vi "Read_Pong.vi"(8 "error in (no error)":errorcluster, 9 "rx state":T1, 10 "result":T2, 11 "TLS connection":refnum<k5>) -> (0 "error out":errorcluster)   [LabVIEW 2021, in "CANsub_API.lvlib"]
doc: "API private: sends a WebSocket pong (opcode 10, same payload) when the last read had a ping (ping len = 0); payload from C_RX_State.ping. Loop-safe: no allocation except W7’s frame (pings are rare)."
uses:
  CANsub_API.lvlib
  CANsub_C.lvlib
  C_Decode_Result.ctl
  C_RX_State.ctl
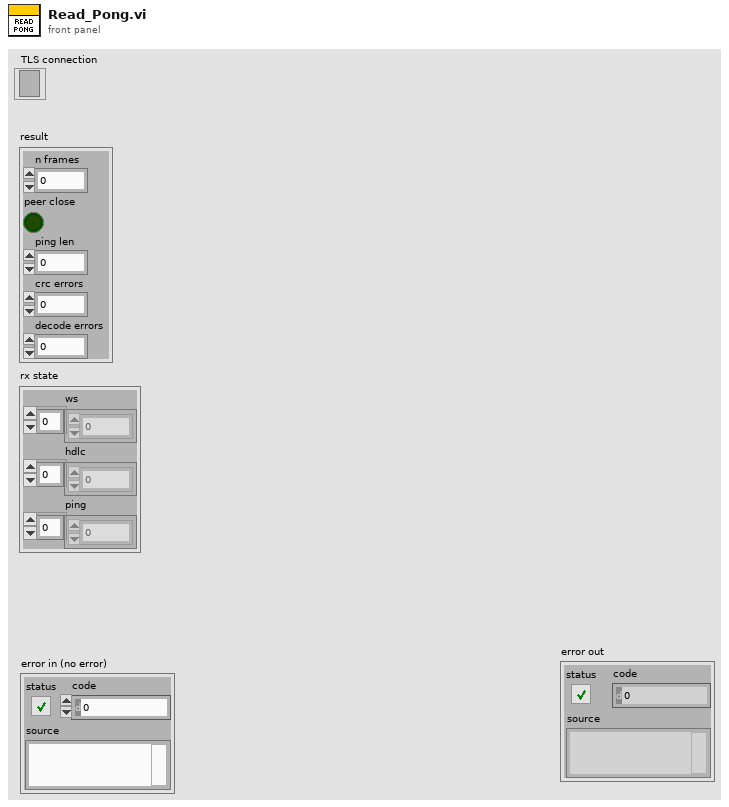
[diagram p1: front panel]
types:
  T1 = typedef "CANsub_C.lvlib/C_RX_State.ctl" = cluster{"ws":u8[], "hdlc":u8[], "ping":u8[]}
  T2 = typedef "CANsub_C.lvlib/C_Decode_Result.ctl" = cluster{"n frames":i32, "peer close":bool, "ping len":i32, "crc errors":u32, "decode errors":i32}
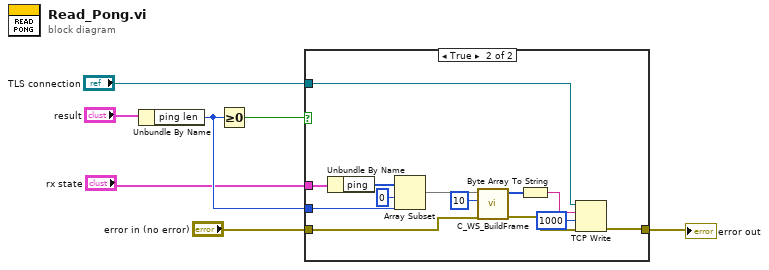
[diagram p0: block diagram]
diagram:
  n1 = Unbundle By Name("result") -> ("ping len"=w3:i32)
  n2 = Greater Or Equal To 0?(x=w3) -> (x >= 0?=w6:bool)
  n3 = case shown="True" w6 {
    tunnel: [w8 w9] -> w5
    tunnel: "error in (no error)" -> [w8 w15]
    tunnel: "rx state" -> [_ w21]
    tunnel: w3 -> [_ w18]
    tunnel: "TLS connection" -> [_ w11]
    frame False {
    }
    frame True {
      n4 = Unbundle By Name(w21) -> ("ping"=w20:u8[])
      n5 = Array Subset(array=w20, index=0, length=w18) -> (w17:u8[])
      n6 = call "C_WS_BuildFrame.vi"("error in (no error)"=w15, "opcode"=u8 10, "payload"=w17) -> ("error out"=w13:errorcluster, "frame"=w14:u8[])  [unwired: 7 in]
      n7 = Byte Array To String(unsigned byte array=w14) -> (string=w12:string)
      n8 = TCP Write(connection ID=w11, data in=w12, error in (no error)=w13, 9:1000 ("timeout ms (25000)")) -> (error out=w9:errorcluster)  [unwired: 2 out]
    }
  }
  "error out" <- w5
